vi "Test MQTT-6.0.0-1.vi"(8 "error in (no error)":errorcluster, 11 "Connection":refnum<class "Connection.lvclass">) -> (0 "error out":errorcluster, 3 "Connection":refnum<class "Connection.lvclass">)   [LabVIEW 2013]
uses:
  <vilib>/LabVIEW Open Source Project/Connection/Connection/Connection.lvclass
  <vilib>/LabVIEW Open Source Project/MQTT Control Packets/Control Packets/ControlPacket/Control Packet Type -- enum.ctl
  <vilib>/LabVIEW Open Source Project/MQTT Control Packets/Control Packets/ControlPacket/QualityOfService -- enum.ctl
  <vilib>/LabVIEW Open Source Project/Connection/Connection.Websockets/Connection.WS.lvclass
  <vilib>/addons/_JKI Toolkits/Caraya/classes/Test/Test.lvclass
  <vilib>/LabVIEW Open Source Project/MQTT Control Packets/Control Packets/CONNECT/CONNECT.lvclass
  <vilib>/LabVIEW Open Source Project/MQTT Control Packets/Control Packets/PUBLISH/PUBLISH.lvclass
  <vilib>/LabVIEW Open Source Project/MQTT Control Packets/Control Packets/ControlPacket/ControlPacket.lvclass
  <vilib>/addons/_JKI Toolkits/Caraya/classes/Assert/Assert.lvclass
panel:
  out "connected":bool
  out "timed out":bool
  out "Should not receive Puback":T1
  out "Connack Packet received?":T1
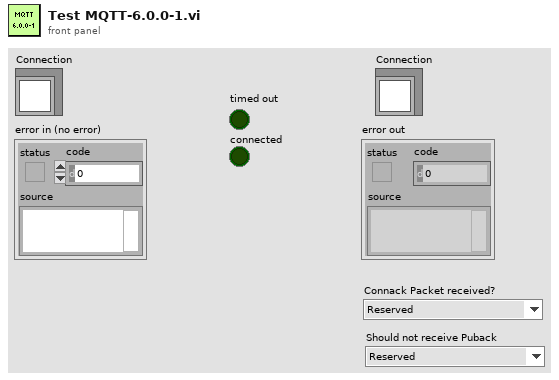
[diagram p1: front panel]
types:
  T1 = typedef "MQTT_Control_Packets.lvlib/ControlPacket.lvclass/Control Packet Type -- enum.ctl" = enum16{"Reserved", "CONNECT", "CONNACK", "PUBLISH", "PUBACK", "PUBREC", "PUBREL", "PUBCOMP", "SUBSCRIBE", "SUBACK", "UNSUBSCRIBE", "UNSUBACK", "PINGREQ", "PINGRESP", "DISCONNECT", "AUTH"}
  T2 = typedef "MQTT_Control_Packets.lvlib/ControlPacket.lvclass/QualityOfService -- enum.ctl" = enum16{"0 (At Most Once)", "1 (At Least Once)", "2 (Exactly Once)"}
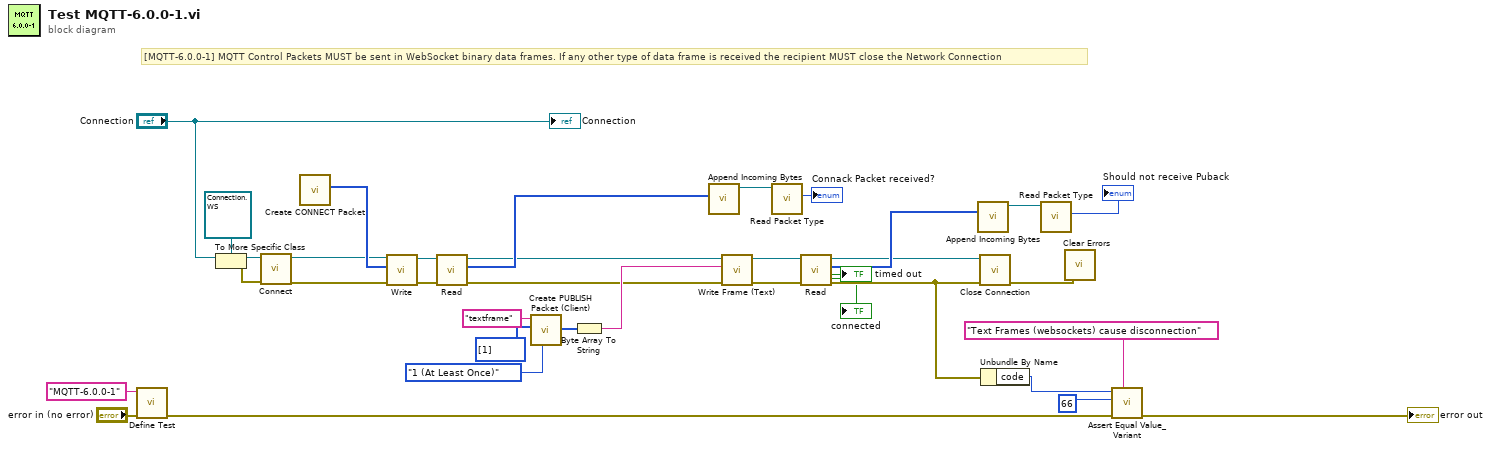
[diagram p0: block diagram]
diagram:
  # "[MQTT-6.0.0-1] MQTT Control Packets MUST be sent in WebSocket binary data frames. If any other type of data frame is received the recipient MUST close the Network Connection"
  n1 = call <vilib>:"Define Test.vi"("error in (no error)"="error in (no error)", "Label (VI Title)"="MQTT-6.0.0-1") -> ("error out"=w31:errorcluster)  [unwired: 9 in]
  n2 = To More Specific Class(target class=refnum<class "Connection.WS.lvclass"> refnum ("Connection.WS in"), reference="Connection") -> (specific class reference=w15:refnum<class "Connection.WS.lvclass">, error out=w1:errorcluster)  [unwired: 1 in]
  n3 = call <vilib>:"Connect.vi"("error in (no error)"=w1, "Connection in"=w15) -> ("error out"=w19:errorcluster, "Connection out"=w3:refnum<class "Connection.WS.lvclass">)  [unwired: 8 in]
  n4 = call <vilib>:"Create CONNECT Packet.vi"() -> ("Bytes Stream"=w20:u8[])  [unwired: 9 in, 2 out]
  n5 = call <vilib>:"Write.vi"("error in (no error)"=w19, "Bytes"=w20, "Connection in"=w3) -> ("error out"=w18:errorcluster, "Connection"=w17:refnum<class "Connection.WS.lvclass">)  [unwired: 7 in]
  n6 = call <vilib>:"Read.vi"("error in (no error)"=w18, "TCPConnection in"=w17) -> ("error out"=w4:errorcluster, "Bytes"=w16:u8[], "TCPConnection out"=w8:refnum<class "Connection.WS.lvclass">)  [unwired: 5 in, 2 out]
  n7 = call <vilib>:"Create PUBLISH Packet (Client).vi"("QoS"=QualityOfService_--_enum."1 (At Least Once)", "Payload"=u8[] [1], "Topic Name"="textframe") -> ("Bytes Stream"=w29:u8[])  [unwired: 5 in, 3 out]
  n8 = Byte Array To String(unsigned byte array=w29) -> (string=w7:string)
  n9 = call <vilib>:"Append Incoming Bytes.vi"("Incoming Packets"=w16) -> ("ControlPacket"=w28:refnum<class "ControlPacket.lvclass">)  [unwired: 7 in, 3 out]
  n10 = call <vilib>:"Write Frame (Text).vi"("error in (no error)"=w4, "Text"=w7, "Connection.WS"=w8) -> ("error out"=w5:errorcluster, "Connection.WS"=w6:refnum<class "Connection.WS.lvclass">)  [unwired: 7 in]
  n11 = call <vilib>:"Read Packet Type.vi"("ControlPacket in"=w28) -> ("Control Packet Type"=→"Connack Packet received?":T1)  [unwired: 9 in, 1 out]
  n12 = call <vilib>:"Read.vi"("error in (no error)"=w5, "TCPConnection in"=w6) -> ("error out"=w12:errorcluster, "timed out"=→"timed out":bool, "Bytes"=w14:u8[], "TCPConnection out"=w13:refnum<class "Connection.WS.lvclass">, "connected"=→"connected":bool)  [unwired: 5 in]
  n13 = call <vilib>:"Append Incoming Bytes.vi"("Incoming Packets"=w14) -> ("ControlPacket"=w26:refnum<class "ControlPacket.lvclass">)  [unwired: 7 in, 3 out]
  n14 = call <vilib>:"Close Connection.vi"("error in (no error)"=w12, "Connection in"=w13) -> ("error out"=w11:errorcluster)  [unwired: 8 in, 1 out]
  n15 = Unbundle By Name(w12) -> ("code"=w24:i32)
  n16 = call <vilib>:"Read Packet Type.vi"("ControlPacket in"=w26) -> ("Control Packet Type"=→"Should not receive Puback":T1)  [unwired: 9 in, 1 out]
  n17 = call <vilib>:"Clear Errors.vi"("error in (no error)"=w11) -> ()  [unwired: 6 in, 1 out]
  n18 = call <vilib>:"Assert Equal Value_Variant.vi"("Label"="Text Frames (websockets) cause disconnection", "error in (no error)"=w31, "Y"=66 ("code"), "X"=w24) -> ("error out"=→"error out":errorcluster)  [unwired: 7 in]
  "Connection" <- "Connection"
